vi "Update Publisher Blackboard Info.vi"(6 "Topic":string, 7 "Blackboard Reference":T1 {"refnum" format="%.0x"}, 8 "error in (no error)":errorcluster, 9 "Blackboard name":string="my_blackboard", 10 "Plugin name":string="my_blackboard", 11 "CIF_Iceoryx_BB in":refnum<class "CIF_Iceoryx_BB.lvclass">) -> (0 "error out":errorcluster, 2 "Full Topic Name":string, 3 "CIF_Iceoryx_BB out":refnum<class "CIF_Iceoryx_BB.lvclass">)   [LabVIEW 2021, in "CIF_Iceoryx_BB.lvclass"]
uses:
  CIF_Iceoryx_BB.lvclass
  <vilib>/CIF Foundation/CIF Iceoryx/Refnum/Typedef/BB Refnum.ctl
  CIF_Iceoryx_BB.lvclass/CIF_Iceoryx_BB.ctl
  Iceorxy Utilities/Iceoryx Channel Utilities.lvlib
  <vilib>/CIF Foundation/CIF Iceoryx/Iceoryx.lvlib
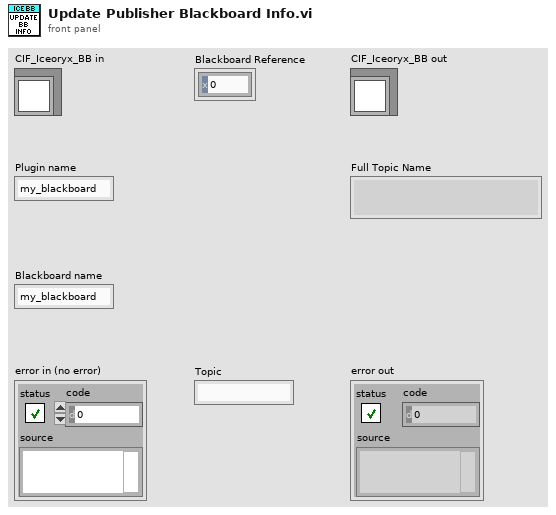
[diagram p1: front panel]
types:
  T1 = typedef "Iceoryx.lvlib/BB Refnum.ctl" = cluster{"refnum":u64, "BB":enum8{"bb"}}
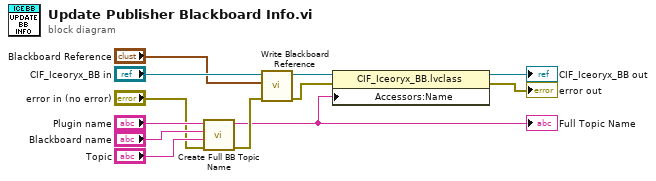
[diagram p0: block diagram]
diagram:
  n1 = call "Create Full BB Topic Name.vi"("error in"="error in (no error)", "Topic"="Topic", "Blackboard name"="Blackboard name", "Plugin name"="Plugin name") -> ("error out"=w6:errorcluster, "String"=w4:string)  [unwired: 6 in]
  "Full Topic Name" <- w4
  n2 = call "Write Blackboard Reference.vi"("error in (no error)"=w6, "BB Refnum"="Blackboard Reference", "CIF_Iceoryx_BB in"="CIF_Iceoryx_BB in") -> ("error out"=w3:errorcluster, "CIF_Iceoryx_BB out"=w5:refnum<class "CIF_Iceoryx_BB.lvclass">)  [unwired: 7 in]
  n3 = property class="CIF_Iceoryx_BB.lvclass"(reference=w5, error in=w3, "Accessors:Name"=w4) -> (reference out=→"CIF_Iceoryx_BB out":refnum<class "CIF_Iceoryx_BB.lvclass">, error out=→"error out":errorcluster)
